vi "RFH-add-create-Permittivity_files_for_all_methods.vi"() -> ()   [LabVIEW 2020, in "RFH-Reflection_File_Handler.lvlib"]
doc: "Run by hand: reads the files of a data folder and saves the permittivity of each calculation method of RDC-permittivity_collection to a destination folder. The user picks the folders and the air/open, DI water, salt water and short files."
uses:
  RFH-Reflection_File_Handler.lvlib
  Computation/RDC-perm_calc_type.ctl
  Computation/RDC-Reflection_Data_Computation.lvlib
panel:
  in  "destination path":path=path "C:/projects/Universitet/Master/data/mastermeasurement/method"
  in  "short":path=path "C:/projects/Universitet/Master/data/Simulated data/Other/complete/100M/sim-P1-short.s2p"
  in  "Salt water":path=path "C:/projects/Universitet/Master/data/Simulated data/Saltwater/complete/100M/sim-P1-saltwater-22p5c.s2p"
  in  "Di water":path=path "C:/projects/Universitet/Master/data/Simulated data/Water/complete/100M/sim-P1-DI_water-22p5c.s2p"
  in  "air/open":path=path "C:/projects/Universitet/Master/data/Simulated data/Other/complete/100M/sim-P1-open.s2p"
  in  "datapath":path=path "C:/projects/Universitet/Master/data/mastermeasurement/converted/22p5c/aff"
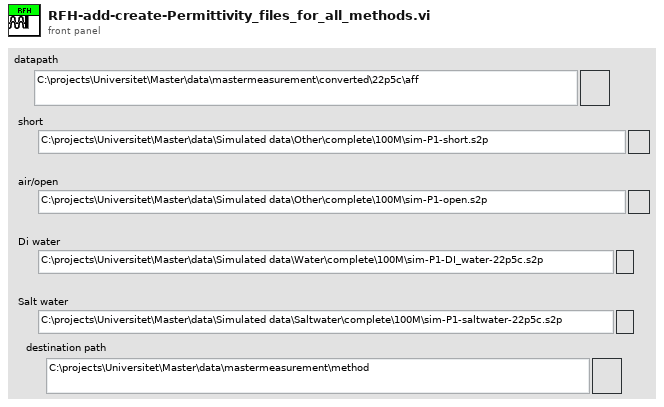
[diagram p1: front panel]
types:
  T1 = typedef "RDC-Reflection_Data_Computation.lvlib/RDC-perm_calc_type.ctl" = enum16{"Basic", "Capacative", "Advance", "Bilinear", "Size"}
  T2 = typedef "RFH-Reflection_File_Handler.lvlib/RFH-common_data_format.ctl" = cluster{"Frequency":dbl[], "Reflection'":dbl[], "Reflection''":dbl[], "Permativity'":dbl[], "Permativity''":dbl[], "Conductivity":dbl[], "Loss Tangent":dbl[], "Resistance":dbl[], "Reactance":dbl[]}
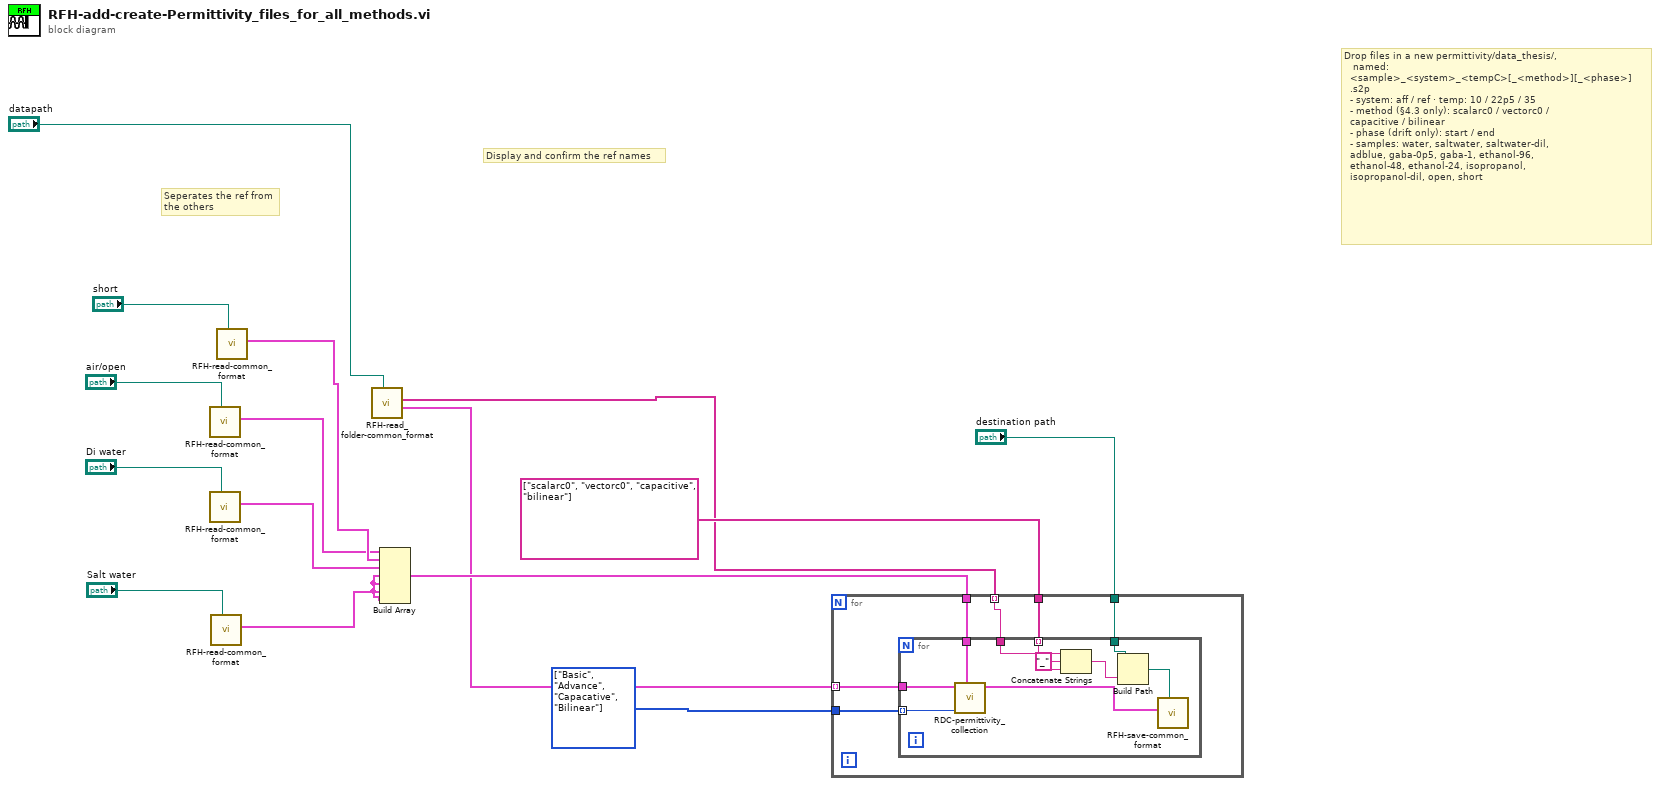
[diagram p0: block diagram]
diagram:
  w4 = T1[] [enum."Basic", enum."Advance", enum."Capacative", enum."Bilinear"] items=["Basic", "Capacative", "Advance", "Bilinear", "Size"] ("Array")
  # "Drop files in a new permittivity/data_thesis/,\n   named:\n  <sample>_<system>_<tempC>[_<method>][_<phase>]\n  .s2p\n  - system: aff / ref · temp: 10 / 22p5 / 35\n  - method (§4.3 only): scalarc0 / vectorc0 /\n  capacitive / bilinear\n  - phase (drift only): start / end\n  - samples: water, saltwater, saltwater-dil,\n  adblue, gaba-0p5, gaba-1, ethanol-96,\n  ethanol-48, ethanol-24, isopropanol,\n  isopropanol-dil, open, short"
  # "Display and confirm the ref names"
  # "Seperates the ref from\nthe others"
  n1 = call "RFH-read-common_format.vi"("file path (dialog if empty)"="air/open") -> ("Common Format"=w6:T2)  [unwired: 9 in, 1 out]
  n2 = call "RFH-read-common_format.vi"("file path (dialog if empty)"="Di water") -> ("Common Format"=w11:T2)  [unwired: 9 in, 1 out]
  n3 = call "RFH-read-common_format.vi"("file path (dialog if empty)"="Salt water") -> ("Common Format"=w5:T2)  [unwired: 9 in, 1 out]
  n4 = call "RFH-read-common_format.vi"("file path (dialog if empty)"="short") -> ("Common Format"=w7:T2)  [unwired: 9 in, 1 out]
  n5 = call "RFH-read_folder-common_format.vi"("File Path"="datapath") -> ("Data"=w8:T2[], "Names"=w2:string[])  [unwired: 8 in, 1 out]
  n6 = Build Array(w6, w7, w11, w5, w5, w5, w5) -> (w9:T2[])
  n7 = for {
    tunnel: w9 -> [w21]
    tunnel: w8 -> [w20] mode=indexing
    tunnel: w4 -> [w19]
    tunnel: string[] ["scalarc0", "vectorc0", "capacitive", "bilinear"] -> [w18]
    tunnel: w2 -> [w17] mode=indexing
    tunnel: "destination path" -> [w16]
    n8 = for {
      tunnel: w21 -> [w31]
      tunnel: w20 -> [w30]
      tunnel: w19 -> [w29] mode=indexing
      tunnel: w18 -> [w24] mode=indexing
      tunnel: w17 -> [w25]
      tunnel: w16 -> [w28]
      n9 = call "RDC-permittivity_collection.vi"("basic data(open, short, water)"=w31, "Perm calc type"=w29, "Common Format"=w30) -> ("Common Format 2"=w26:T2)  [unwired: 8 in]
      n10 = Concatenate Strings(w25, "_" ("string"), w24) -> (w22:string)
      n11 = Build Path(base path=w28, name or relative path=w22) -> (appended path=w27:path)
      n12 = call "RFH-save-common_format.vi"("file path (use dialog)"=w27, "Common Format"=w26) -> ()  [unwired: 9 in, 1 out]
    }
  }
